vi "Find Method By Signature.vi"(8 "error in":errorcluster, 9 "Parameter Types":refnum<k24>[](array[refnum]), 10 "Method Name":string, 11 "Declaring Type in":refnum<k24>) -> (0 "error out":errorcluster, 2 "Method Info":refnum<k24>, 3 "Declaring Type out":refnum<k24>)   [LabVIEW 2026, in "ToastNotification.lvlib" / "Reflection DotNet.lvlib"]
doc: "Resolve a public method by name and exact parameter types using System.Type.GetMethod(String, Type[]). Skipped on incoming error. Borrow Declaring Type and Parameter Types. Caller owns Method Info; Declaring Type out is only an alias. A missing method can return null and must not be treated as a valid MethodInfo."
uses:
  Reflection DotNet.lvlib
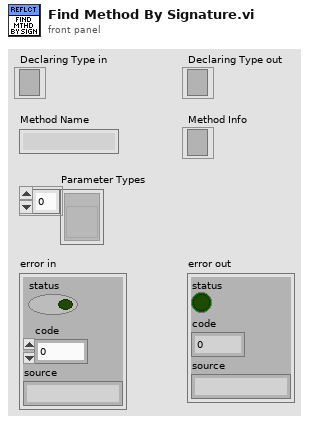
[diagram p1: front panel]
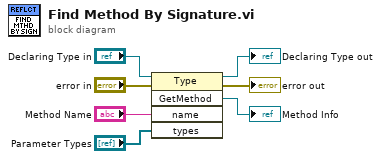
[diagram p0: block diagram]
diagram:
  n1 = invoke class="Type" method="GetMethod"(reference="Declaring Type in", error in="error in", "name"="Method Name", "types"="Parameter Types") -> (reference out=→"Declaring Type out":refnum<k24>, error out=→"error out":errorcluster, "GetMethod"=→"Method Info":refnum<k24>)  [unwired: 1 in, 2 out]
